vi "NEO Set PID Coefficients.vi"(6 "error in":errorcluster, 7 "Closed Loop Slot":T1 items=["Slot 0", "Slot 1", "Slot 2", "Slot 3"], 8 "PID Gains":T2, 9 "Spark refnum":T3) -> (0 "error out":errorcluster, 3 "Spark refnum out":T3)   [LabVIEW 2027]
uses:
  <vilib>/REV Custom Controls/REVSparkRefnum.ctl
  <resource>/objmgr/REVSpark.rc
  <vilib>/REVLibDriver/REVLibDriver.lvlib
  <vilib>/REV Custom Controls/SPARK Closed Loop Slot.ctl
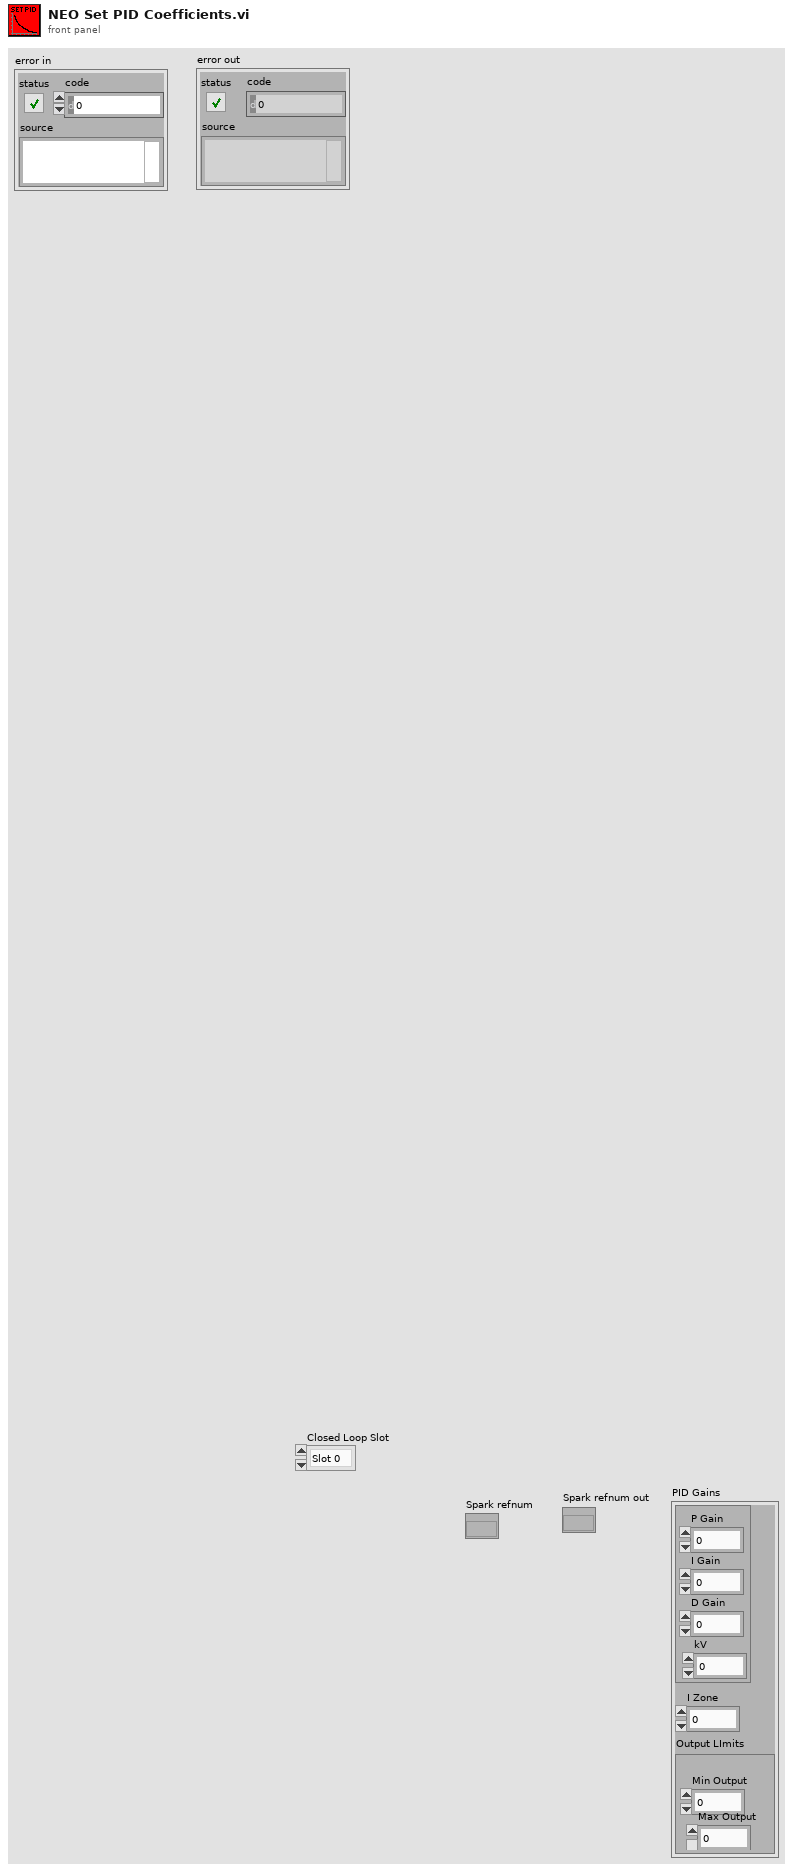
[diagram p1: front panel]
types:
  T1 = typedef "SPARK Closed Loop Slot.ctl" = u16
  T2 = cluster{cluster{"P Gain":dbl, "I Gain":dbl, "D Gain":dbl, "kV":dbl}, "I Zone":dbl, "Output LImits":cluster{"Min Output":dbl, "Max Output":dbl}}
  T3 = typedef "REVLibDriver.lvlib/REVSparkRefnum.ctl" = refnum<k20>
  T4 = cluster{"P Gain":dbl, "I Gain":dbl, "D Gain":dbl, "kV":dbl}
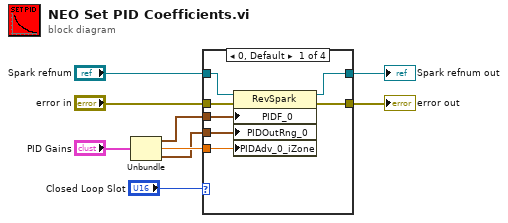
[diagram p0: block diagram]
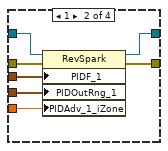
[diagram p2: hidden frame]
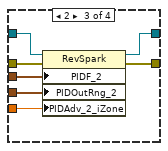
[diagram p3: hidden frame]
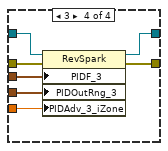
[diagram p4: hidden frame]
diagram:
  n1 = Unbundle("PID Gains") -> (w7:T4, "I Zone"=w5:dbl, "Output LImits"=w4:cluster{"Min Output":dbl, "Max Output":dbl})
  n2 = case shown="0, Default" "Closed Loop Slot" {
    tunnel: "Spark refnum" -> [w16 w23 w30 w37]
    tunnel: w7 -> [w14 w22 w29 w36]
    tunnel: "error in" -> [w15 w21 w28 w35]
    tunnel: w5 -> [w12 w20 w27 w34]
    tunnel: w4 -> [w13 w19 w26 w33]
    tunnel: [w11 w18 w25 w32] -> w3
    tunnel: [w10 w17 w24 w31] -> w2
    frame 0, Default {
      n3 = property class="RevSpark"(reference=w16, error in=w15, "PIDF_0"=w14, "PIDOutRng_0"=w13, "PIDAdv_0_iZone"=w12) -> (reference out=w11:T3, error out=w10:errorcluster)
    }
    frame 1 {
      n4 = property class="RevSpark"(reference=w23, error in=w21, "PIDF_1"=w22, "PIDOutRng_1"=w19, "PIDAdv_1_iZone"=w20) -> (reference out=w18:T3, error out=w17:errorcluster)
    }
    frame 2 {
      n5 = property class="RevSpark"(reference=w30, error in=w28, "PIDF_2"=w29, "PIDOutRng_2"=w26, "PIDAdv_2_iZone"=w27) -> (reference out=w25:T3, error out=w24:errorcluster)
    }
    frame 3 {
      n6 = property class="RevSpark"(reference=w37, error in=w35, "PIDF_3"=w36, "PIDOutRng_3"=w33, "PIDAdv_3_iZone"=w34) -> (reference out=w32:T3, error out=w31:errorcluster)
    }
  }
  "error out" <- w2
  "Spark refnum out" <- w3
